vi "[ex ce] Integration.vi"() -> ()   [LabVIEW 2021]
doc: "CE-Math example.\n\n::: CalcExpress Toolkit :::\nCopyright (c) 2000-2026 Konstantin Shifershteyn. All rights reserved."
uses:
  ce exmpl - 1D difference info.ctl
  <vilib>/gmath/NI_Gmath.lvlib
panel:
  out "max relative difference":T1={"index"=-1, "absolute difference"=0.0, "relative difference, %"=0.0} {"relative difference, %" format="%#.6g"; "absolute difference" format="%#.6g"}
  out "max absolute difference":T1={"index"=-1, "absolute difference"=0.0, "relative difference, %"=0.0} {"relative difference, %" format="%#.6g"; "absolute difference" format="%#.6g"}
  in  "formula info":cluster{"formula":string, "x-variable":string}={"formula"="sinc(x)+sin(2*x)+sin(3*x)+sin(2*x*x)", "x-variable"="x"}
  in  "end":dbl=10.0 format="%.2f"
  in  "start":dbl format="%.2f"
  out "speed ratio":dbl format="%.3f"
  out "GM ticks":u32 caption="ms"
  out "CE ticks":u32 caption="ms"
  out "CE Graph":cluster{"x":dbl[], "f(x)":dbl[]}[](graph) caption="CalcExpress"
  out "GM Graph":cluster{"x":dbl[], "f(x)":dbl[]}[](graph) caption="G Math"
  # "NOTE    CalcExpress uses (^) operator to perform bitwise-XOR operation but not exponentiation operation.\nYou have to use double-asterisk (**) operator to compute an exponent in a CalcExpress expression. For sample, x**y ."
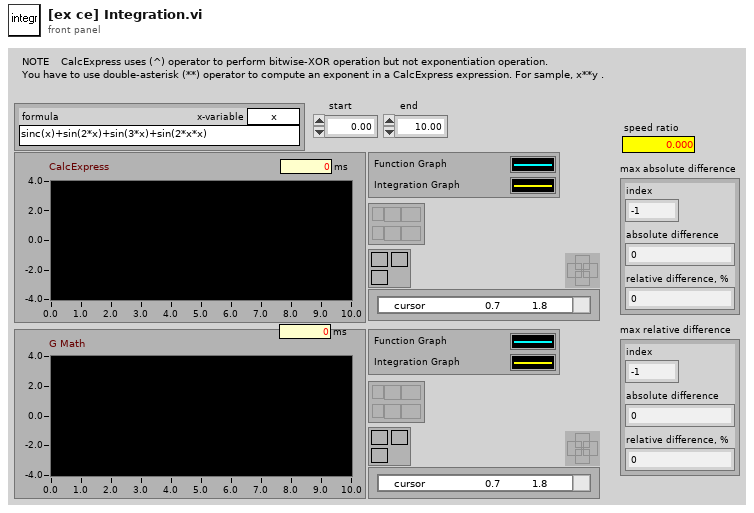
[diagram p1: front panel]
types:
  T1 = typedef "ce exmpl - 1D difference info.ctl" = cluster{"index":i32, "absolute difference":dbl, "relative difference, %":dbl}
  T2 = cluster{"X Values":dbl[], "Integral of Y":dbl[]}[]
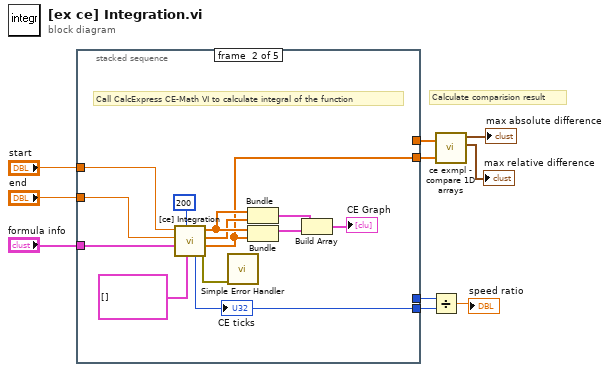
[diagram p0: block diagram]
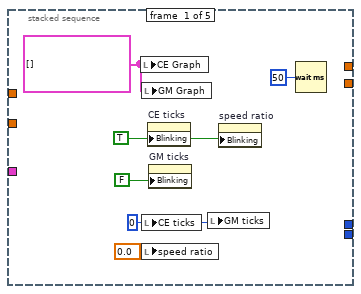
[diagram p2: hidden frame]
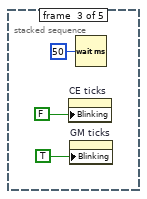
[diagram p3: hidden frame]
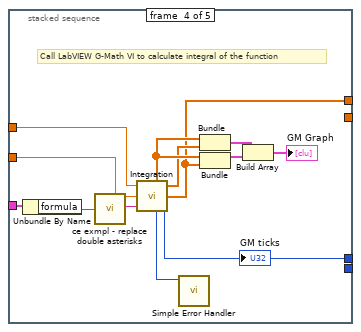
[diagram p4: hidden frame]
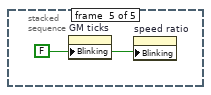
[diagram p5: hidden frame]
diagram:
  # "Calculate comparision result"
  n1 = stacked-sequence {
    tunnel: "start" -> [_ w27 _ w42 _]
    tunnel: "end" -> [_ w26 _ w43 _]
    tunnel: "formula info" -> [_ w25 _ w41 _]
    tunnel: [_ w28 _ _ _] -> w10
    tunnel: [_ _ _ w44 _] -> w8
    tunnel: [_ _ _ w35 _] -> w4
    tunnel: [_ w19 _ _ _] -> w3
    frame #0 {
      w11 = cluster{"x":dbl[], "f(x)":dbl[]}[] [] ("CE Graph")
      w13 = u32 0 ("CE ticks")
      w15 = TRUE ("Write Attribute")
      n2 = local write "CE Graph"(w11) -> ()
      n3 = local write "GM Graph"(w11) -> ()
      n4 = local write "CE ticks"(w13) -> ()
      n5 = local write "speed ratio"(0.0 ("speed ratio")) -> ()
      n6 = property on="CE ticks" class="DigNum (strict)"("Blinking"=w15) -> ()  [unwired: 2 in, 2 out]
      n7 = property on="GM ticks" class="DigNum (strict)"("Blinking"=FALSE ("Write Attribute")) -> ()  [unwired: 2 in, 2 out]
      n8 = local write "GM ticks"(w13) -> ()
      n9 = property on="speed ratio" class="DigNum (strict)"("Blinking"=w15) -> ()  [unwired: 2 in, 2 out]
      n10 = Wait (ms)(milliseconds to wait=u32 50) -> ()  [unwired: 1 out]
    }
    frame #1 {
      # "Call CalcExpress CE-Math VI to calculate integral of the function"
      n11 = call "[ce] Integration.vi"("parameters"=cluster{"name":string, "value":dbl}[] [] ("additional parameters"), "# points"=200, "formula info"=w25, "end"=w26, "start"=w27) -> ("error out"=w29:errorcluster, "Integral of Y"=w19:dbl[], "Y Values"=w21:dbl[], "X Values"=w22:dbl[], "ticks"=w28:u32)  [unwired: 2 in]
      "CE ticks" <- w28
      n12 = call <vilib>:"Simple Error Handler.vi"("error in (no error)"=w29) -> ()  [unwired: 4 in, 5 out]
      n13 = Bundle("X Values"=w22, "Y Values"=w21) -> (w24:cluster{"X Values":dbl[], "Y Values":dbl[]})  [unwired: 1 in]
      n14 = Bundle("X Values"=w22, "Integral of Y"=w19) -> (w23:cluster{"X Values":dbl[], "Integral of Y":dbl[]})  [unwired: 1 in]
      n15 = Build Array(w24, w23) -> (→"CE Graph":T2)
    }
    frame #2 {
      n16 = property on="CE ticks" class="DigNum (strict)"("Blinking"=FALSE ("Write Attribute")) -> ()  [unwired: 2 in, 2 out]
      n17 = property on="GM ticks" class="DigNum (strict)"("Blinking"=TRUE ("Write Attribute")) -> ()  [unwired: 2 in, 2 out]
      n18 = Wait (ms)(milliseconds to wait=u32 50) -> ()  [unwired: 1 out]
    }
    frame #3 {
      # "Call LabVIEW G-Math VI to calculate integral of the function"
      n19 = Unbundle By Name(w41) -> ("formula"=w33:string)
      n20 = call "ce exmpl - replace double asterisks .vi"("formula in"=w33) -> ("formula out"=w34:string)  [unwired: 4 in]
      n21 = call <vilib>:"Integration.vi"("formula"=w34, "end"=w43, "start"=w42) -> ("ticks"=w44:u32, "error"=w45:i32, "Integral of Y"=w35:dbl[], "Y Values"=w38:dbl[], "X Values"=w39:dbl[])
      "GM ticks" <- w44
      n22 = call <vilib>:"Simple Error Handler.vi"("error code (no error:0)"=w45) -> ()  [unwired: 4 in, 5 out]
      n23 = Bundle("X Values"=w39, "Y Values"=w38) -> (w37:cluster{"X Values":dbl[], "Y Values":dbl[]})  [unwired: 1 in]
      n24 = Bundle("X Values"=w39, "Integral of Y"=w35) -> (w36:cluster{"X Values":dbl[], "Integral of Y":dbl[]})  [unwired: 1 in]
      n25 = Build Array(w37, w36) -> (→"GM Graph":T2)
    }
    frame #4 {
      w46 = FALSE ("Write Attribute")
      n26 = property on="GM ticks" class="DigNum (strict)"("Blinking"=w46) -> ()  [unwired: 2 in, 2 out]
      n27 = property on="speed ratio" class="DigNum (strict)"("Blinking"=w46) -> ()  [unwired: 2 in, 2 out]
    }
  }
  n28 = Divide(x=w8, y=w10) -> (x/y=→"speed ratio":dbl)
  n29 = call "ce exmpl - compare 1D arrays.vi"("checking array B"=w3, "standard array A"=w4) -> ("max relative difference"=→"max relative difference":T1, "max absolute difference"=→"max absolute difference":T1)  [unwired: 1 in, 2 out]
